vi "Open-Close.vi"(5 "Username":string, 6 "Password":string, 7 "Address":string, 8 "Error In":errorcluster) -> (0 "Error Out":errorcluster)   [LabVIEW 2018, in "Tests.lvlib" / "SFTP Directory.lvlib"]
uses:
  SFTP Directory.lvlib
  src/Toolkit/SFTP Directory/Support/Open from SFTP.vi
  src/Toolkit/SFTP Directory/Support/Close to SFTP.vi
  <vilib>/addons/_JKI Toolkits/Caraya/classes/Test/Test.lvclass
  <vilib>/addons/_JKI Toolkits/Caraya/classes/Assert/Assert.lvclass
  src/Toolkit/SFTP Directory/SFTP Directory.lvclass
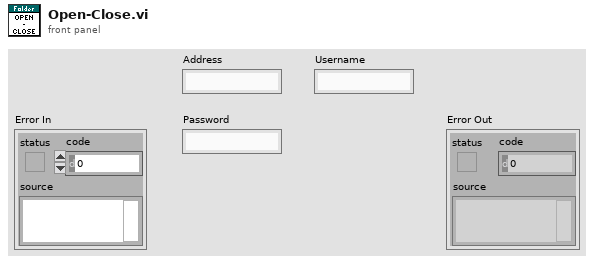
[diagram p1: front panel]
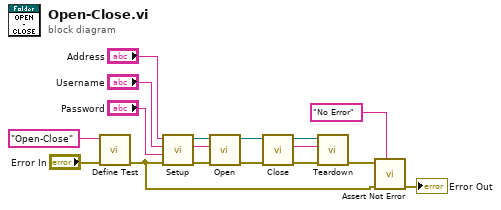
[diagram p0: block diagram]
diagram:
  n1 = call <vilib>:"Define Test.vi"("error in (no error)"="Error In", "Label (VI Title)"="Open-Close") -> ("error out"=w13:errorcluster)  [unwired: 9 in]
  n2 = call "Setup.vi"("Error In"=w13, "Password"="Password", "Username"="Username", "Address"="Address") -> ("Error Out"=w3:errorcluster, "Temporary Directory"=w2:string, "SFTP"=w4:refnum<class "SFTP.lvclass">)  [unwired: 5 in]
  n3 = call-poly "Open.vi"("Error In"=w3, "Remote Path"=w2, "SFTP"=w4) -> ("Error Out"=w12:errorcluster, "SFTP Directory"=w11:refnum<class "SFTP Directory.lvclass">)  [unwired: 7 in]
  n4 = call-poly "Close.vi"("Error In"=w12, "SFTP Directory"=w11) -> ("Error Out"=w10:errorcluster, "Remote Path"=w1:string, "SFTP"=w5:refnum<class "SFTP.lvclass">)  [unwired: 7 in]
  n5 = call "Teardown.vi"("Error In"=w10, "Temporary Directory"=w1, "SFTP"=w5) -> ("Error Out"=w9:errorcluster)  [unwired: 8 in]
  n6 = call <vilib>:"Assert Not Error.vi"("Label"="No Error", "error in (no error)"=w13, "Not Error?"=w9) -> ("error out"=→"Error Out":errorcluster)  [unwired: 8 in]
